vi "serialization tests.vi"() -> (0 "serialization error":errorcluster, 3 "channels equal":bool, 4 "validation error":errorcluster)   [LabVIEW 2014, in "TEC tests.lvlib"]
uses:
  TEC tests.lvlib
  configuration/TEC configuration.lvclass/TEC configuration.ctl
  configuration/Read channels.vi
  <vilib>/NI/Tag Bus Module Framework/channel/TBM channel.lvclass
  configuration/TEC configuration.lvclass
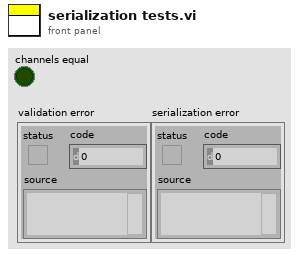
[diagram p1: front panel]
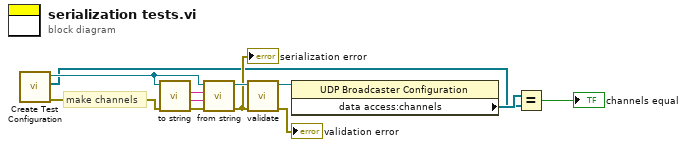
[diagram p0: block diagram]
diagram:
  # "make channels"
  n1 = call "Create Test Configuration.vi"() -> ("error out"=w1:errorcluster, "Array"=w2:refnum<class "TBM channel.lvclass">[], "TEC configuration out"=w3:refnum<class "TEC configuration.lvclass">)  [unwired: 9 in]
  n2 = call-dynamic "to string.vi"("error in"=w1, "TEC configuration in"=w3) -> ("error out"=w12:errorcluster, "data"=w11:string, "version"=w10:string)  [unwired: 6 in, 1 out]
  n3 = call-dynamic "from string.vi"("error in"=w12, "data"=w11, "version"=w10, "TEC configuration in"=w3) -> ("error out"=w7:errorcluster, "TEC configuration out"=w9:refnum<class "TEC configuration.lvclass">)  [unwired: 6 in]
  "serialization error" <- w7
  n4 = call-dynamic "validate.vi"("error in"=w7, "TEC configuration in"=w9) -> ("error out"=→"validation error":errorcluster, "TEC configuration out"=w5:refnum<class "TEC configuration.lvclass">)  [unwired: 8 in]
  n5 = property class="UDP Broadcaster Configuration"(reference=w5) -> ("data access:channels"=w4:refnum<class "TBM channel.lvclass">[])  [unwired: 1 in, 2 out]
  n6 = Equal?(x=w4, y=w2) -> (x = y?=→"channels equal":bool)
